vi "PicoScope6000aExampleStreamingQueue.vi"() -> ()   [LabVIEW 2010]
doc: "ps6000a Streaming example filling a single set of channel buffers at a time with LabVIEW queues."
uses:
  shared/PicoBuffers.ctl
  <vilib>/Waveform/DWDTOps.llb/DWDT Analog to Digital.vi
  PicoScope6000aLib/PicoScope6000aDigitalChannelSettings.ctl
  PicoScope6000aLib/PicoScope6000aAnalogChannelSettings.ctl
  shared/Buffer and Transfer Settings.ctl
panel:
  out "overflow":i16 format="%010b"
  in  "Channels":T1={"Channel A Settings "={"Enabled"=TRUE, "Coupling"=50, "Range"=5, "Analogue Offset"=0.0, "BandWidth"=0}, "Channel B Settings "={"Enabled"=FALSE, "Coupling"=50, "Range"=5, "Analogue Offset"=0.0, "BandWidth"=0}, "Channel C Settings "={"Enabled"=FALSE, "Coupling"=50, "Range"=5, "Analogue Offset"=0.0, "BandWidth"=0}, "Channel D Settings "={"Enabled"=FALSE, "Coupling"=50, "Range"=5, "Analogue Offset"=0.0, "BandWidth"=0}, "Channel E Settings "={"Enabled"=FALSE, "Coupling"=50, "Range"=5, "Analogue Offset"=0.0, "BandWidth"=0}, "Channel F Settings "={"Enabled"=FALSE, "Coupling"=50, "Range"=5, "Analogue Offset"=0.0, "BandWidth"=0}, "Channel G Settings "={"Enabled"=FALSE, "Coupling"=50, "Range"=5, "Analogue Offset"=0.0, "BandWidth"=0}, "Channel H Settings "={"Enabled"=FALSE, "Coupling"=50, "Range"=5, "Analogue Offset"=0.0, "BandWidth"=0}} {"Channel H Settings"."BandWidth" items=["Full"=0, "100kHz"=100000, "20kHz"=200000, "1MHz"=1000000, "20MHz"=20000000, "25MHz"=25000000, "50MHz"=50000000, "200MHz"=200000000, "250MHz"=250000000, "500MHz"=500000000]; "Channel H Settings"."Range" items=["10mV"=0, "20mV"=1, "50mV"=2, "100mV"=3, "200mV"=4, "500mV"=5, "1V"=6, "2V"=7, "5V"=8, "10V"=9, "20V"=10, "50V"=11, "100V"=12, "200V"=13, "x10_Probe_100mV"=32, "x10_Probe_200mV"=33, "x10_Probe_500mV"=34, "x10_Probe_1V"=35, "x10_Probe_2V"=36, "x10_Probe_5V"=37, "x10_Probe_10V"=38, "x10_Probe_20V"=39, "x10_Probe_50V"=40, "x10_Probe_100V"=41, "x10_Probe_200V"=42, "x10_Probe_500V"=43, "CURRENT_CLAMP_60A_2A"=10500, "CURRENT_CLAMP_60A_5A"=10501, "CURRENT_CLAMP_60A_10A"=10502, "CURRENT_CLAMP_60A_20A"=10503, "CURRENT_CLAMP_60A_50A"=10504, "CURRENT_CLAMP_60A_60A"=10505, "CURRENT_CLAMP_60A_V2_0_5A"=10600, "CURRENT_CLAMP_60A_V2_1A"=10601, "CURRENT_CLAMP_60A_V2_2A"=10602, "CURRENT_CLAMP_60A_V2_5A"=10603, "CURRENT_CLAMP_60A_V2_10A"=10604, "CURRENT_CLAMP_60A_V2_20A"=10605, "CURRENT_CLAMP_60A_V2_50A"=10606, "CURRENT_CLAMP_60A_V2_60A"=10607, "RESISTANCE_LEAD_NEG5_TO_20OHM"=7000, "RESISTANCE_LEAD_NEG50_TO_200OHM"=7001, "RESISTANCE_LEAD_NEG500_TO_2KOHM"=7002, "RESISTANCE_LEAD_NEG5K_TO_20KOHM"=7003, "RESISTANCE_LEAD_NEG50K_TO_LEAD_200KOHM"=7004, "RESISTANCE_LEAD_NEG500K_TO_LEAD_2MOHM"=7005, "RESISTANCE_LEAD_DIODE_TEST"=7006, "HT_NEG3_TO_5KV"=8950, "HT_NEG3_TO_10KV"=8951, "HT_NEG5_TO_20KV"=8952, "HT_NEG5_TO_50KV"=8953, "HT_NEG5_TO_100KV"=8954, "HT_NEG3_TO_5KV_INVERTED"=8955, "HT_NEG3_TO_10KV_INVERTED"=8956, "HT_NEG5_TO_20KV_INVERTED"=8957, "HT_NEG5_TO_50KV_INVERTED"=8958, "HT_NEG5_TO_100KV_INVERTED"=8959, "TEMPERATURE_NEG50_TO_150DEGC"=9000, "PRESSURE_SENSOR_-100k-150k_PASCALS"=9100, "PRESSURE_SENSOR_-100k_TO_400k_PASCALS"=9101, "PRESSURE_SENSOR_-200k_TO_800k_PASCALS"=9102, "PRESSURE_SENSOR_-400k_TO_1600k_PASCALS"=9103, "PRESSURE_SENSOR_-400k_TO_3400k_PASCALS"=9104, "PRESSURE_SENSOR_-150k_TO_1350k_PASCALS"=9105]; "Channel H Settings"."Coupling" items=["AC"=0, "DC 1M Ohm"=1, "DC 50 Ohm"=50]; "Channel G Settings"."BandWidth" items=["Full"=0, "100kHz"=100000, "20kHz"=200000, "1MHz"=1000000, "20MHz"=20000000, "25MHz"=25000000, "50MHz"=50000000, "200MHz"=200000000, "250MHz"=250000000, "500MHz"=500000000]; "Channel G Settings"."Range" items=["10mV"=0, "20mV"=1, "50mV"=2, "100mV"=3, "200mV"=4, "500mV"=5, "1V"=6, "2V"=7, "5V"=8, "10V"=9, "20V"=10, "50V"=11, "100V"=12, "200V"=13, "x10_Probe_100mV"=32, "x10_Probe_200mV"=33, "x10_Probe_500mV"=34, "x10_Probe_1V"=35, "x10_Probe_2V"=36, "x10_Probe_5V"=37, "x10_Probe_10V"=38, "x10_Probe_20V"=39, "x10_Probe_50V"=40, "x10_Probe_100V"=41, "x10_Probe_200V"=42, "x10_Probe_500V"=43, "CURRENT_CLAMP_60A_2A"=10500, "CURRENT_CLAMP_60A_5A"=10501, "CURRENT_CLAMP_60A_10A"=10502, "CURRENT_CLAMP_60A_20A"=10503, "CURRENT_CLAMP_60A_50A"=10504, "CURRENT_CLAMP_60A_60A"=10505, "CURRENT_CLAMP_60A_V2_0_5A"=10600, "CURRENT_CLAMP_60A_V2_1A"=10601, "CURRENT_CLAMP_60A_V2_2A"=10602, "CURRENT_CLAMP_60A_V2_5A"=10603, "CURRENT_CLAMP_60A_V2_10A"=10604, "CURRENT_CLAMP_60A_V2_20A"=10605, "CURRENT_CLAMP_60A_V2_50A"=10606, "CURRENT_CLAMP_60A_V2_60A"=10607, "RESISTANCE_LEAD_NEG5_TO_20OHM"=7000, "RESISTANCE_LEAD_NEG50_TO_200OHM"=7001, "RESISTANCE_LEAD_NEG500_TO_2KOHM"=7002, "RESISTANCE_LEAD_NEG5K_TO_20KOHM"=7003, "RESISTANCE_LEAD_NEG50K_TO_LEAD_200KOHM"=7004, "RESISTANCE_LEAD_NEG500K_TO_LEAD_2MOHM"=7005, "RESISTANCE_LEAD_DIODE_TEST"=7006, "HT_NEG3_TO_5KV"=8950, "HT_NEG3_TO_10KV"=8951, "HT_NEG5_TO_20KV"=8952, "HT_NEG5_TO_50KV"=8953, "HT_NEG5_TO_100KV"=8954, "HT_NEG3_TO_5KV_INVERTED"=8955, "HT_NEG3_TO_10KV_INVERTED"=8956, "HT_NEG5_TO_20KV_INVERTED"=8957, "HT_NEG5_TO_50KV_INVERTED"=8958, "HT_NEG5_TO_100KV_INVERTED"=8959, "TEMPERATURE_NEG50_TO_150DEGC"=9000, "PRESSURE_SENSOR_-100k-150k_PASCALS"=9100, "PRESSURE_SENSOR_-100k_TO_400k_PASCALS"=9101, "PRESSURE_SENSOR_-200k_TO_800k_PASCALS"=9102, "PRESSURE_SENSOR_-400k_TO_1600k_PASCALS"=9103, "PRESSURE_SENSOR_-400k_TO_3400k_PASCALS"=9104, "PRESSURE_SENSOR_-150k_TO_1350k_PASCALS"=9105]; "Channel G Settings"."Coupling" items=["AC"=0, "DC 1M Ohm"=1, "DC 50 Ohm"=50]; "Channel F Settings"."BandWidth" items=["Full"=0, "100kHz"=100000, "20kHz"=200000, "1MHz"=1000000, "20MHz"=20000000, "25MHz"=25000000, "50MHz"=50000000, "200MHz"=200000000, "250MHz"=250000000, "500MHz"=500000000]; "Channel F Settings"."Range" items=["10mV"=0, "20mV"=1, "50mV"=2, "100mV"=3, "200mV"=4, "500mV"=5, "1V"=6, "2V"=7, "5V"=8, "10V"=9, "20V"=10, "50V"=11, "100V"=12, "200V"=13, "x10_Probe_100mV"=32, "x10_Probe_200mV"=33, "x10_Probe_500mV"=34, "x10_Probe_1V"=35, "x10_Probe_2V"=36, "x10_Probe_5V"=37, "x10_Probe_10V"=38, "x10_Probe_20V"=39, "x10_Probe_50V"=40, "x10_Probe_100V"=41, "x10_Probe_200V"=42, "x10_Probe_500V"=43, "CURRENT_CLAMP_60A_2A"=10500, "CURRENT_CLAMP_60A_5A"=10501, "CURRENT_CLAMP_60A_10A"=10502, "CURRENT_CLAMP_60A_20A"=10503, "CURRENT_CLAMP_60A_50A"=10504, "CURRENT_CLAMP_60A_60A"=10505, "CURRENT_CLAMP_60A_V2_0_5A"=10600, "CURRENT_CLAMP_60A_V2_1A"=10601, "CURRENT_CLAMP_60A_V2_2A"=10602, "CURRENT_CLAMP_60A_V2_5A"=10603, "CURRENT_CLAMP_60A_V2_10A"=10604, "CURRENT_CLAMP_60A_V2_20A"=10605, "CURRENT_CLAMP_60A_V2_50A"=10606, "CURRENT_CLAMP_60A_V2_60A"=10607, "RESISTANCE_LEAD_NEG5_TO_20OHM"=7000, "RESISTANCE_LEAD_NEG50_TO_200OHM"=7001, "RESISTANCE_LEAD_NEG500_TO_2KOHM"=7002, "RESISTANCE_LEAD_NEG5K_TO_20KOHM"=7003, "RESISTANCE_LEAD_NEG50K_TO_LEAD_200KOHM"=7004, "RESISTANCE_LEAD_NEG500K_TO_LEAD_2MOHM"=7005, "RESISTANCE_LEAD_DIODE_TEST"=7006, "HT_NEG3_TO_5KV"=8950, "HT_NEG3_TO_10KV"=8951, "HT_NEG5_TO_20KV"=8952, "HT_NEG5_TO_50KV"=8953, "HT_NEG5_TO_100KV"=8954, "HT_NEG3_TO_5KV_INVERTED"=8955, "HT_NEG3_TO_10KV_INVERTED"=8956, "HT_NEG5_TO_20KV_INVERTED"=8957, "HT_NEG5_TO_50KV_INVERTED"=8958, "HT_NEG5_TO_100KV_INVERTED"=8959, "TEMPERATURE_NEG50_TO_150DEGC"=9000, "PRESSURE_SENSOR_-100k-150k_PASCALS"=9100, "PRESSURE_SENSOR_-100k_TO_400k_PASCALS"=9101, "PRESSURE_SENSOR_-200k_TO_800k_PASCALS"=9102, "PRESSURE_SENSOR_-400k_TO_1600k_PASCALS"=9103, "PRESSURE_SENSOR_-400k_TO_3400k_PASCALS"=9104, "PRESSURE_SENSOR_-150k_TO_1350k_PASCALS"=9105]; "Channel F Settings"."Coupling" items=["AC"=0, "DC 1M Ohm"=1, "DC 50 Ohm"=50]; "Channel E Settings"."BandWidth" items=["Full"=0, "100kHz"=100000, "20kHz"=200000, "1MHz"=1000000, "20MHz"=20000000, "25MHz"=25000000, "50MHz"=50000000, "200MHz"=200000000, "250MHz"=250000000, "500MHz"=500000000]; "Channel E Settings"."Range" items=["10mV"=0, "20mV"=1, "50mV"=2, "100mV"=3, "200mV"=4, "500mV"=5, "1V"=6, "2V"=7, "5V"=8, "10V"=9, "20V"=10, "50V"=11, "100V"=12, "200V"=13, "x10_Probe_100mV"=32, "x10_Probe_200mV"=33, "x10_Probe_500mV"=34, "x10_Probe_1V"=35, "x10_Probe_2V"=36, "x10_Probe_5V"=37, "x10_Probe_10V"=38, "x10_Probe_20V"=39, "x10_Probe_50V"=40, "x10_Probe_100V"=41, "x10_Probe_200V"=42, "x10_Probe_500V"=43, "CURRENT_CLAMP_60A_2A"=10500, "CURRENT_CLAMP_60A_5A"=10501, "CURRENT_CLAMP_60A_10A"=10502, "CURRENT_CLAMP_60A_20A"=10503, "CURRENT_CLAMP_60A_50A"=10504, "CURRENT_CLAMP_60A_60A"=10505, "CURRENT_CLAMP_60A_V2_0_5A"=10600, "CURRENT_CLAMP_60A_V2_1A"=10601, "CURRENT_CLAMP_60A_V2_2A"=10602, "CURRENT_CLAMP_60A_V2_5A"=10603, "CURRENT_CLAMP_60A_V2_10A"=10604, "CURRENT_CLAMP_60A_V2_20A"=10605, "CURRENT_CLAMP_60A_V2_50A"=10606, "CURRENT_CLAMP_60A_V2_60A"=10607, "RESISTANCE_LEAD_NEG5_TO_20OHM"=7000, "RESISTANCE_LEAD_NEG50_TO_200OHM"=7001, "RESISTANCE_LEAD_NEG500_TO_2KOHM"=7002, "RESISTANCE_LEAD_NEG5K_TO_20KOHM"=7003, "RESISTANCE_LEAD_NEG50K_TO_LEAD_200KOHM"=7004, "RESISTANCE_LEAD_NEG500K_TO_LEAD_2MOHM"=7005, "RESISTANCE_LEAD_DIODE_TEST"=7006, "HT_NEG3_TO_5KV"=8950, "HT_NEG3_TO_10KV"=8951, "HT_NEG5_TO_20KV"=8952, "HT_NEG5_TO_50KV"=8953, "HT_NEG5_TO_100KV"=8954, "HT_NEG3_TO_5KV_INVERTED"=8955, "HT_NEG3_TO_10KV_INVERTED"=8956, "HT_NEG5_TO_20KV_INVERTED"=8957, "HT_NEG5_TO_50KV_INVERTED"=8958, "HT_NEG5_TO_100KV_INVERTED"=8959, "TEMPERATURE_NEG50_TO_150DEGC"=9000, "PRESSURE_SENSOR_-100k-150k_PASCALS"=9100, "PRESSURE_SENSOR_-100k_TO_400k_PASCALS"=9101, "PRESSURE_SENSOR_-200k_TO_800k_PASCALS"=9102, "PRESSURE_SENSOR_-400k_TO_1600k_PASCALS"=9103, "PRESSURE_SENSOR_-400k_TO_3400k_PASCALS"=9104, "PRESSURE_SENSOR_-150k_TO_1350k_PASCALS"=9105]; "Channel E Settings"."Coupling" items=["AC"=0, "DC 1M Ohm"=1, "DC 50 Ohm"=50]; "Channel D Settings"."BandWidth" items=["Full"=0, "100kHz"=100000, "20kHz"=200000, "1MHz"=1000000, "20MHz"=20000000, "25MHz"=25000000, "50MHz"=50000000, "200MHz"=200000000, "250MHz"=250000000, "500MHz"=500000000]; "Channel D Settings"."Range" items=["10mV"=0, "20mV"=1, "50mV"=2, "100mV"=3, "200mV"=4, "500mV"=5, "1V"=6, "2V"=7, "5V"=8, "10V"=9, "20V"=10, "50V"=11, "100V"=12, "200V"=13, "x10_Probe_100mV"=32, "x10_Probe_200mV"=33, "x10_Probe_500mV"=34, "x10_Probe_1V"=35, "x10_Probe_2V"=36, "x10_Probe_5V"=37, "x10_Probe_10V"=38, "x10_Probe_20V"=39, "x10_Probe_50V"=40, "x10_Probe_100V"=41, "x10_Probe_200V"=42, "x10_Probe_500V"=43, "CURRENT_CLAMP_60A_2A"=10500, "CURRENT_CLAMP_60A_5A"=10501, "CURRENT_CLAMP_60A_10A"=10502, "CURRENT_CLAMP_60A_20A"=10503, "CURRENT_CLAMP_60A_50A"=10504, "CURRENT_CLAMP_60A_60A"=10505, "CURRENT_CLAMP_60A_V2_0_5A"=10600, "CURRENT_CLAMP_60A_V2_1A"=10601, "CURRENT_CLAMP_60A_V2_2A"=10602, "CURRENT_CLAMP_60A_V2_5A"=10603, "CURRENT_CLAMP_60A_V2_10A"=10604, "CURRENT_CLAMP_60A_V2_20A"=10605, "CURRENT_CLAMP_60A_V2_50A"=10606, "CURRENT_CLAMP_60A_V2_60A"=10607, "RESISTANCE_LEAD_NEG5_TO_20OHM"=7000, "RESISTANCE_LEAD_NEG50_TO_200OHM"=7001, "RESISTANCE_LEAD_NEG500_TO_2KOHM"=7002, "RESISTANCE_LEAD_NEG5K_TO_20KOHM"=7003, "RESISTANCE_LEAD_NEG50K_TO_LEAD_200KOHM"=7004, "RESISTANCE_LEAD_NEG500K_TO_LEAD_2MOHM"=7005, "RESISTANCE_LEAD_DIODE_TEST"=7006, "HT_NEG3_TO_5KV"=8950, "HT_NEG3_TO_10KV"=8951, "HT_NEG5_TO_20KV"=8952, "HT_NEG5_TO_50KV"=8953, "HT_NEG5_TO_100KV"=8954, "HT_NEG3_TO_5KV_INVERTED"=8955, "HT_NEG3_TO_10KV_INVERTED"=8956, "HT_NEG5_TO_20KV_INVERTED"=8957, "HT_NEG5_TO_50KV_INVERTED"=8958, "HT_NEG5_TO_100KV_INVERTED"=8959, "TEMPERATURE_NEG50_TO_150DEGC"=9000, "PRESSURE_SENSOR_-100k-150k_PASCALS"=9100, "PRESSURE_SENSOR_-100k_TO_400k_PASCALS"=9101, "PRESSURE_SENSOR_-200k_TO_800k_PASCALS"=9102, "PRESSURE_SENSOR_-400k_TO_1600k_PASCALS"=9103, "PRESSURE_SENSOR_-400k_TO_3400k_PASCALS"=9104, "PRESSURE_SENSOR_-150k_TO_1350k_PASCALS"=9105]; "Channel D Settings"."Coupling" items=["AC"=0, "DC 1M Ohm"=1, "DC 50 Ohm"=50]; "Channel C Settings"."BandWidth" items=["Full"=0, "100kHz"=100000, "20kHz"=200000, "1MHz"=1000000, "20MHz"=20000000, "25MHz"=25000000, "50MHz"=50000000, "200MHz"=200000000, "250MHz"=250000000, "500MHz"=500000000]; "Channel C Settings"."Range" items=["10mV"=0, "20mV"=1, "50mV"=2, "100mV"=3, "200mV"=4, "500mV"=5, "1V"=6, "2V"=7, "5V"=8, "10V"=9, "20V"=10, "50V"=11, "100V"=12, "200V"=13, "x10_Probe_100mV"=32, "x10_Probe_200mV"=33, "x10_Probe_500mV"=34, "x10_Probe_1V"=35, "x10_Probe_2V"=36, "x10_Probe_5V"=37, "x10_Probe_10V"=38, "x10_Probe_20V"=39, "x10_Probe_50V"=40, "x10_Probe_100V"=41, "x10_Probe_200V"=42, "x10_Probe_500V"=43, "CURRENT_CLAMP_60A_2A"=10500, "CURRENT_CLAMP_60A_5A"=10501, "CURRENT_CLAMP_60A_10A"=10502, "CURRENT_CLAMP_60A_20A"=10503, "CURRENT_CLAMP_60A_50A"=10504, "CURRENT_CLAMP_60A_60A"=10505, "CURRENT_CLAMP_60A_V2_0_5A"=10600, "CURRENT_CLAMP_60A_V2_1A"=10601, "CURRENT_CLAMP_60A_V2_2A"=10602, "CURRENT_CLAMP_60A_V2_5A"=10603, "CURRENT_CLAMP_60A_V2_10A"=10604, "CURRENT_CLAMP_60A_V2_20A"=10605, "CURRENT_CLAMP_60A_V2_50A"=10606, "CURRENT_CLAMP_60A_V2_60A"=10607, "RESISTANCE_LEAD_NEG5_TO_20OHM"=7000, "RESISTANCE_LEAD_NEG50_TO_200OHM"=7001, "RESISTANCE_LEAD_NEG500_TO_2KOHM"=7002, "RESISTANCE_LEAD_NEG5K_TO_20KOHM"=7003, "RESISTANCE_LEAD_NEG50K_TO_LEAD_200KOHM"=7004, "RESISTANCE_LEAD_NEG500K_TO_LEAD_2MOHM"=7005, "RESISTANCE_LEAD_DIODE_TEST"=7006, "HT_NEG3_TO_5KV"=8950, "HT_NEG3_TO_10KV"=8951, "HT_NEG5_TO_20KV"=8952, "HT_NEG5_TO_50KV"=8953, "HT_NEG5_TO_100KV"=8954, "HT_NEG3_TO_5KV_INVERTED"=8955, "HT_NEG3_TO_10KV_INVERTED"=8956, "HT_NEG5_TO_20KV_INVERTED"=8957, "HT_NEG5_TO_50KV_INVERTED"=8958, "HT_NEG5_TO_100KV_INVERTED"=8959, "TEMPERATURE_NEG50_TO_150DEGC"=9000, "PRESSURE_SENSOR_-100k-150k_PASCALS"=9100, "PRESSURE_SENSOR_-100k_TO_400k_PASCALS"=9101, "PRESSURE_SENSOR_-200k_TO_800k_PASCALS"=9102, "PRESSURE_SENSOR_-400k_TO_1600k_PASCALS"=9103, "PRESSURE_SENSOR_-400k_TO_3400k_PASCALS"=9104, "PRESSURE_SENSOR_-150k_TO_1350k_PASCALS"=9105]; "Channel C Settings"."Coupling" items=["AC"=0, "DC 1M Ohm"=1, "DC 50 Ohm"=50]; "Channel B Settings"."BandWidth" items=["Full"=0, "100kHz"=100000, "20kHz"=200000, "1MHz"=1000000, "20MHz"=20000000, "25MHz"=25000000, "50MHz"=50000000, "200MHz"=200000000, "250MHz"=250000000, "500MHz"=500000000]; "Channel B Settings"."Range" items=["10mV"=0, "20mV"=1, "50mV"=2, "100mV"=3, "200mV"=4, "500mV"=5, "1V"=6, "2V"=7, "5V"=8, "10V"=9, "20V"=10, "50V"=11, "100V"=12, "200V"=13, "x10_Probe_100mV"=32, "x10_Probe_200mV"=33, "x10_Probe_500mV"=34, "x10_Probe_1V"=35, "x10_Probe_2V"=36, "x10_Probe_5V"=37, "x10_Probe_10V"=38, "x10_Probe_20V"=39, "x10_Probe_50V"=40, "x10_Probe_100V"=41, "x10_Probe_200V"=42, "x10_Probe_500V"=43, "CURRENT_CLAMP_60A_2A"=10500, "CURRENT_CLAMP_60A_5A"=10501, "CURRENT_CLAMP_60A_10A"=10502, "CURRENT_CLAMP_60A_20A"=10503, "CURRENT_CLAMP_60A_50A"=10504, "CURRENT_CLAMP_60A_60A"=10505, "CURRENT_CLAMP_60A_V2_0_5A"=10600, "CURRENT_CLAMP_60A_V2_1A"=10601, "CURRENT_CLAMP_60A_V2_2A"=10602, "CURRENT_CLAMP_60A_V2_5A"=10603, "CURRENT_CLAMP_60A_V2_10A"=10604, "CURRENT_CLAMP_60A_V2_20A"=10605, "CURRENT_CLAMP_60A_V2_50A"=10606, "CURRENT_CLAMP_60A_V2_60A"=10607, "RESISTANCE_LEAD_NEG5_TO_20OHM"=7000, "RESISTANCE_LEAD_NEG50_TO_200OHM"=7001, "RESISTANCE_LEAD_NEG500_TO_2KOHM"=7002, "RESISTANCE_LEAD_NEG5K_TO_20KOHM"=7003, "RESISTANCE_LEAD_NEG50K_TO_LEAD_200KOHM"=7004, "RESISTANCE_LEAD_NEG500K_TO_LEAD_2MOHM"=7005, "RESISTANCE_LEAD_DIODE_TEST"=7006, "HT_NEG3_TO_5KV"=8950, "HT_NEG3_TO_10KV"=8951, "HT_NEG5_TO_20KV"=8952, "HT_NEG5_TO_50KV"=8953, "HT_NEG5_TO_100KV"=8954, "HT_NEG3_TO_5KV_INVERTED"=8955, "HT_NEG3_TO_10KV_INVERTED"=8956, "HT_NEG5_TO_20KV_INVERTED"=8957, "HT_NEG5_TO_50KV_INVERTED"=8958, "HT_NEG5_TO_100KV_INVERTED"=8959, "TEMPERATURE_NEG50_TO_150DEGC"=9000, "PRESSURE_SENSOR_-100k-150k_PASCALS"=9100, "PRESSURE_SENSOR_-100k_TO_400k_PASCALS"=9101, "PRESSURE_SENSOR_-200k_TO_800k_PASCALS"=9102, "PRESSURE_SENSOR_-400k_TO_1600k_PASCALS"=9103, "PRESSURE_SENSOR_-400k_TO_3400k_PASCALS"=9104, "PRESSURE_SENSOR_-150k_TO_1350k_PASCALS"=9105]; "Channel B Settings"."Coupling" items=["AC"=0, "DC 1M Ohm"=1, "DC 50 Ohm"=50]; "Channel A Settings"."Range" items=["10mV"=0, "20mV"=1, "50mV"=2, "100mV"=3, "200mV"=4, "500mV"=5, "1V"=6, "2V"=7, "5V"=8, "10V"=9, "20V"=10, "50V"=11, "100V"=12, "200V"=13, "x10_Probe_100mV"=32, "x10_Probe_200mV"=33, "x10_Probe_500mV"=34, "x10_Probe_1V"=35, "x10_Probe_2V"=36, "x10_Probe_5V"=37, "x10_Probe_10V"=38, "x10_Probe_20V"=39, "x10_Probe_50V"=40, "x10_Probe_100V"=41, "x10_Probe_200V"=42, "x10_Probe_500V"=43, "CURRENT_CLAMP_60A_2A"=10500, "CURRENT_CLAMP_60A_5A"=10501, "CURRENT_CLAMP_60A_10A"=10502, "CURRENT_CLAMP_60A_20A"=10503, "CURRENT_CLAMP_60A_50A"=10504, "CURRENT_CLAMP_60A_60A"=10505, "CURRENT_CLAMP_60A_V2_0_5A"=10600, "CURRENT_CLAMP_60A_V2_1A"=10601, "CURRENT_CLAMP_60A_V2_2A"=10602, "CURRENT_CLAMP_60A_V2_5A"=10603, "CURRENT_CLAMP_60A_V2_10A"=10604, "CURRENT_CLAMP_60A_V2_20A"=10605, "CURRENT_CLAMP_60A_V2_50A"=10606, "CURRENT_CLAMP_60A_V2_60A"=10607, "RESISTANCE_LEAD_NEG5_TO_20OHM"=7000, "RESISTANCE_LEAD_NEG50_TO_200OHM"=7001, "RESISTANCE_LEAD_NEG500_TO_2KOHM"=7002, "RESISTANCE_LEAD_NEG5K_TO_20KOHM"=7003, "RESISTANCE_LEAD_NEG50K_TO_LEAD_200KOHM"=7004, "RESISTANCE_LEAD_NEG500K_TO_LEAD_2MOHM"=7005, "RESISTANCE_LEAD_DIODE_TEST"=7006, "HT_NEG3_TO_5KV"=8950, "HT_NEG3_TO_10KV"=8951, "HT_NEG5_TO_20KV"=8952, "HT_NEG5_TO_50KV"=8953, "HT_NEG5_TO_100KV"=8954, "HT_NEG3_TO_5KV_INVERTED"=8955, "HT_NEG3_TO_10KV_INVERTED"=8956, "HT_NEG5_TO_20KV_INVERTED"=8957, "HT_NEG5_TO_50KV_INVERTED"=8958, "HT_NEG5_TO_100KV_INVERTED"=8959, "TEMPERATURE_NEG50_TO_150DEGC"=9000, "PRESSURE_SENSOR_-100k-150k_PASCALS"=9100, "PRESSURE_SENSOR_-100k_TO_400k_PASCALS"=9101, "PRESSURE_SENSOR_-200k_TO_800k_PASCALS"=9102, "PRESSURE_SENSOR_-400k_TO_1600k_PASCALS"=9103, "PRESSURE_SENSOR_-400k_TO_3400k_PASCALS"=9104, "PRESSURE_SENSOR_-150k_TO_1350k_PASCALS"=9105]; "Channel A Settings"."BandWidth" items=["Full"=0, "100kHz"=100000, "20kHz"=200000, "1MHz"=1000000, "20MHz"=20000000, "25MHz"=25000000, "50MHz"=50000000, "200MHz"=200000000, "250MHz"=250000000, "500MHz"=500000000]; "Channel A Settings"."Coupling" items=["AC"=0, "DC 1M Ohm"=1, "DC 50 Ohm"=50]}
  out "Triggered":bool
  out "triggerAt":u64
  in  "Poll Delay %":dbl=1.0 format="%#_13g"
  in  "Poll Holdoff %":dbl=33.0 format="%#_13g"
  out "Port 0":digitalwaveform(graph)={"t0"=timestamp(0 s since 1904-01-01), "dt"=1.004800013071339e-06, "Y"={"transitions"=[], "data"=[]}}
  out "Analog Channels":cluster{i32, dbl, "Data":dbl[]}[](graph)
  in  "Write to TDMS file":bool
  out "Queue depth":i32(graph)
  out "queue depth":i32
  in  "Data file":path=path "PicoScope6000aExampleStreaming Data"
  out "Max ADC value":i16
  out "DownSample Interval (sec)":dbl=1.0000000130088963e-06 format="%#.5p"
  out "Chunk time":u32
  out "Elapsed time":dbl
  in  "Auto Stop":bool
  in  "Apply Settings":bool
  in  "Digital Channels":T2={"Port 0 Settings "={"Enabled"=FALSE, "Hysteresis"=3, "Threshold Level (Volts)"=[1.0, 1.0, 1.0, 1.0, 1.0, 1.0, 1.0, 1.0]}, "Port 1 Settings"={"Enabled"=FALSE, "Hysteresis"=3, "Threshold Level (Volts)"=[1.0, 1.0, 1.0, 1.0, 1.0, 1.0, 1.0, 1.0]}} {"Port 1 Settings"."Threshold Level (Volts)" format="%#_4p"; "Port 1 Settings"."Hysteresis" items=["PICO_VERY_HIGH_400MV", "PICO_HIGH_200MV", "PICO_NORMAL_100MV", "PICO_LOW_50MV"]; "Port 0 Settings"."Threshold Level (Volts)" format="%#_4p"; "Port 0 Settings"."Hysteresis" items=["PICO_VERY_HIGH_400MV", "PICO_HIGH_200MV", "PICO_NORMAL_100MV", "PICO_LOW_50MV"]}
  in  "No of Buffers":i32=2 min=2
  in  "Streaming Acquisition Settings":T3={"preTriggerSamples"=0, "postTriggerSamples"=1000000, "Requested sampleInterval"=100.0, "sampleIntervalTimeUnits"=2} {"sampleIntervalTimeUnits" items=["femtoseconds", "picoseconds", "nanoseconds", "microseconds", "millseconds", "seconds"]; "postTriggerSamples" format="%_6p"; "preTriggerSamples" format="%_6p"}
  in  "Buffer and Transfer Settings":T4={"startIndex"=0, "Samples"=1000000, "Down Sample Ratio"=1, "Down-Sample Mode"=2147483648} {"Down-Sample Mode" items=["RAW none"=2147483648, "None"=0, "Aggregate"=1, "Decimate"=2, "Average"=4]; "Down Sample Ratio" step=1; "Samples" format="%_6p"}
  in  "Trigger Settings":T5={"Trigger Enabled"=FALSE, "Trigger Threshold (Volts)"=0.0, "Trigger Direction"=2, "Trigger Delay (samples)"=0, "Auto Trigger Time (us)"=100000, "Trigger Source"=0} {"Trigger Source" items=["Channel A"=0, "Channel B"=1, "Channel C"=2, "Channel D"=3, "Channel E"=4, "Channel F"=5, "Channel G"=6, "Channel H"=7, "Port 0"=128, "Port 1"=129, "Trigger AUX"=1001]; "Trigger Direction" items=["Rising"=2, "Falling"=3]; "Trigger Threshold (Volts)" format="%#_6p"}
  in  "stop":bool
  out "Device Info":T6
  out "Pico 6000a Units":string
  in  "Resolution":u32(ring) items=["8-bit"=0, "12-bit"=1, "14-bit"=2, "15-bit"=3, "16-bit"=4, "10-bit"=10]
  in  "Serial Number":string
  in  "Use Serial Number":bool
  in  "error in (no error)":errorcluster
  # "LSB ChA"
  # "D8-D15"
  # "DO-D7"
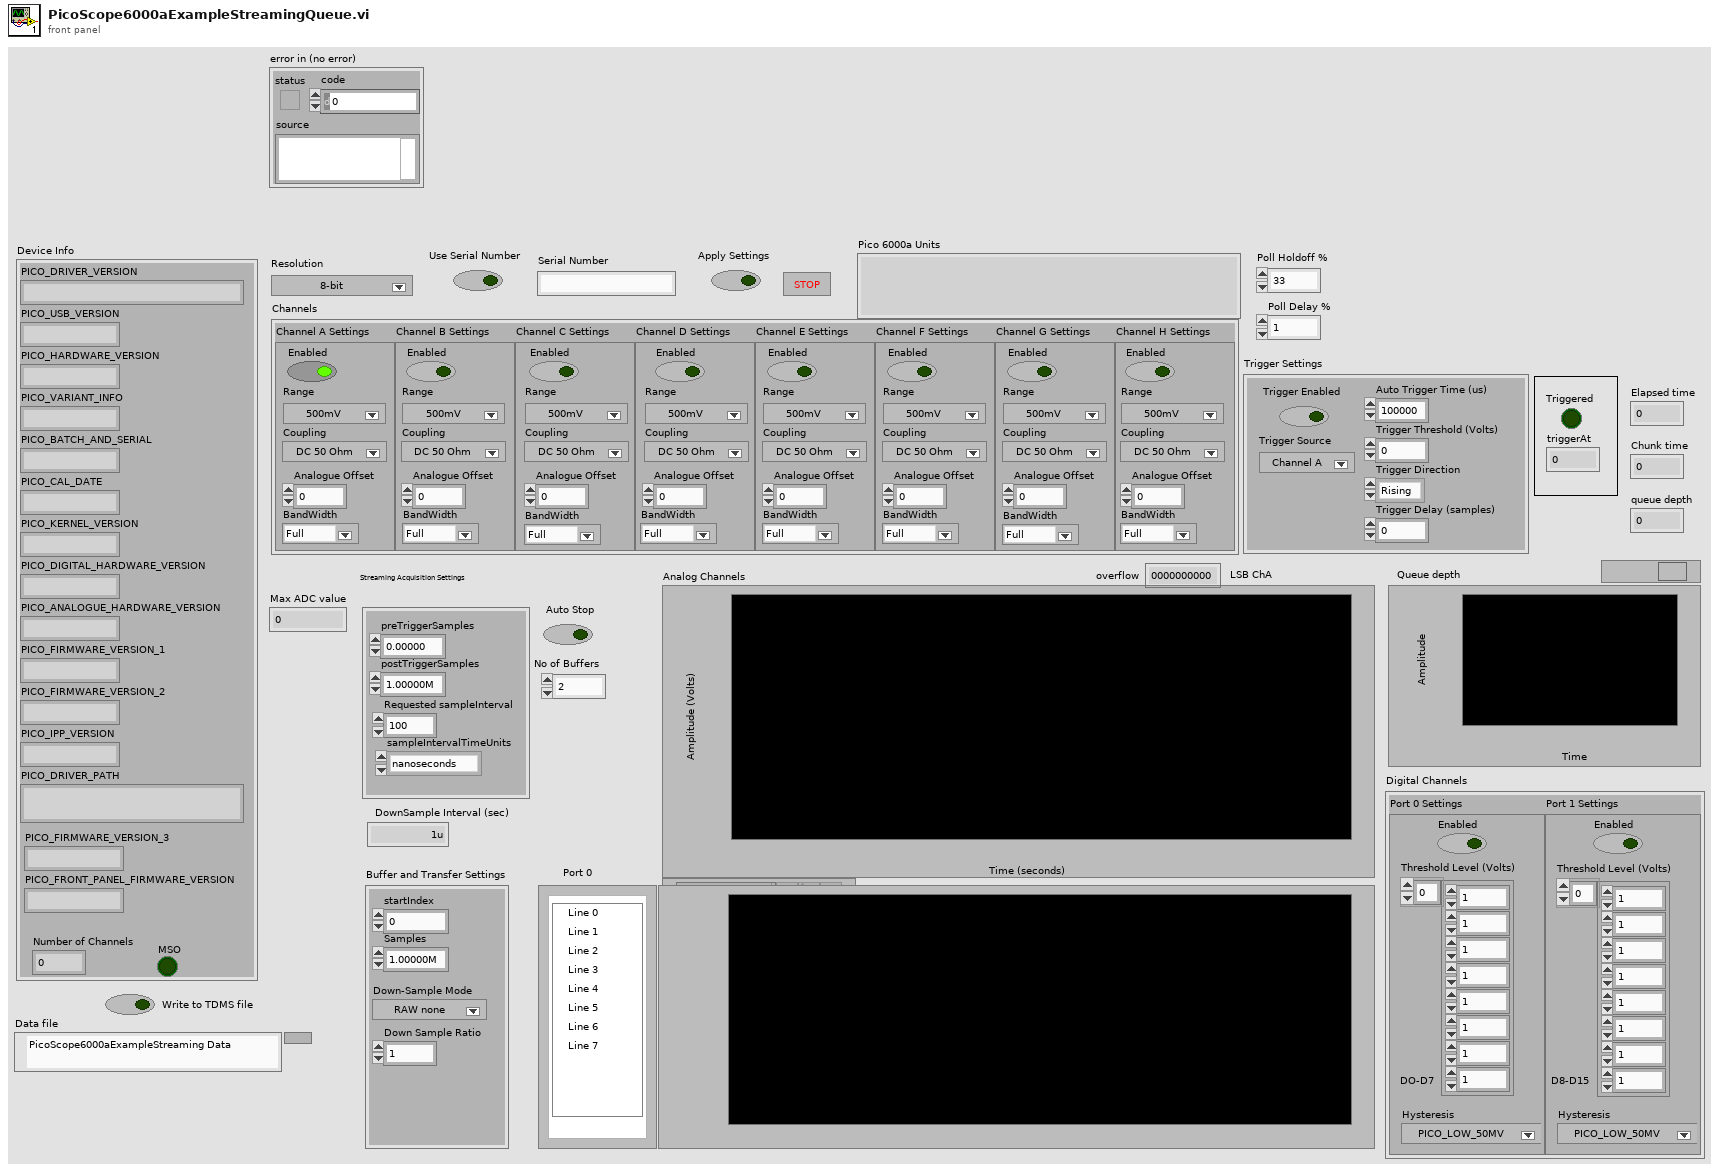
[diagram p1: front panel]
types:
  T1 = typedef "PicoScope6000aAnalogChannelSettings.ctl" = cluster{"Channel A Settings ":cluster{"Enabled":bool, "Coupling":i16, "Range":u32, "Analogue Offset":dbl, "BandWidth":u32}, "Channel B Settings ":cluster{"Enabled":bool, "Coupling":i16, "Range":u32, "Analogue Offset":dbl, "BandWidth":u32}, "Channel C Settings ":cluster{"Enabled":bool, "Coupling":i16, "Range":u32, "Analogue Offset":dbl, "BandWidth":u32}, "Channel D Settings ":cluster{"Enabled":bool, "Coupling":i16, "Range":u32, "Analogue Offset":dbl, "BandWidth":u32}, "Channel E Settings ":cluster{"Enabled":bool, "Coupling":i16, "Range":u32, "Analogue Offset":dbl, "BandWidth":u32}, "Channel F Settings ":cluster{"Enabled":bool, "Coupling":i16, "Range":u32, "Analogue Offset":dbl, "BandWidth":u32}, "Channel G Settings ":cluster{"Enabled":bool, "Coupling":i16, "Range":u32, "Analogue Offset":dbl, "BandWidth":u32}, "Channel H Settings ":cluster{"Enabled":bool, "Coupling":i16, "Range":u32, "Analogue Offset":dbl, "BandWidth":u32}}
  T2 = typedef "PicoScope6000aDigitalChannelSettings.ctl" = cluster{"Port 0 Settings ":cluster{"Enabled":bool, "Hysteresis":u32, "Threshold Level (Volts)":dbl[]}, "Port 1 Settings":cluster{"Enabled":bool, "Hysteresis":u32, "Threshold Level (Volts)":dbl[]}}
  T3 = cluster{"preTriggerSamples":u64, "postTriggerSamples":u64, "Requested sampleInterval":dbl, "sampleIntervalTimeUnits":u32}
  T4 = typedef "Buffer and Transfer Settings.ctl" = cluster{"startIndex":u64, "Samples":u64, "Down Sample Ratio":u64, "Down-Sample Mode":u32}
  T5 = cluster{"Trigger Enabled":bool, "Trigger Threshold (Volts)":dbl, "Trigger Direction":u16, "Trigger Delay (samples)":u64, "Auto Trigger Time (us)":u32, "Trigger Source":u32}
  T6 = cluster{"PICO_DRIVER_VERSION":string, "PICO_USB_VERSION":string, "PICO_HARDWARE_VERSION":string, "PICO_VARIANT_INFO":string, "PICO_BATCH_AND_SERIAL":string, "PICO_CAL_DATE":string, "PICO_KERNEL_VERSION":string, "PICO_DIGITAL_HARDWARE_VERSION":string, "PICO_ANALOGUE_HARDWARE_VERSION":string, "PICO_FIRMWARE_VERSION_1":string, "PICO_FIRMWARE_VERSION_2":string, "PICO_IPP_VERSION":string, "PICO_DRIVER_PATH":string, "PICO_FIRMWARE_VERSION_3":string, "PICO_FRONT_PANEL_FIRMWARE_VERSION":string, "Number of Channels":i16, "MSO":bool}
  T7 = typedef "PicoBuffers.ctl" = cluster{"Max Buffer Pointers":u64[][][], "Min Buffer Pointers":u64[][][], "StreamingDataInfo":cluster{"Channel":u32, "Down-Sample Mode":u32, "PICO_DATA_TYPE":enum32{"PICO_INT8_T", "PICO_INT16_T", "PICO_INT32_T", "PICO_UINT32_T", "PICO_INT64_T", ""}, "Samples":i32, "bufferIndex":u64, "startIndex":i32, "overflow":i16}[][]}
  T8 = enum16{"open", "open or create", "create or replace", "create", "open (read-only)"}
  T9 = cluster{"sampleInterval":dbl, "sampleIntervalTimeUnits":u32}
  T10 = cluster{"triggerAt":u64, "triggered":bool, "autoStop":bool}
  T11 = cluster{"Channel A Buffer":i16[], "Channel B Buffer":i16[], "Channel C Buffer":i16[], "Channel D Buffer":i16[], "Channel E Buffer":i16[], "Channel F Buffer":i16[], "Channel G Buffer":i16[], "Channel H Buffer":i16[], "Port 0 Buffer":i16[], "Port 1 Buffer":i16[]}
  T12 = cluster{"Channel":u32, "Down-Sample Mode":u32, "PICO_DATA_TYPE":enum32{"PICO_INT8_T", "PICO_INT16_T", "PICO_INT32_T", "PICO_UINT32_T", "PICO_INT64_T", ""}, "Samples":i32, "bufferIndex":u64, "startIndex":i32, "overflow":i16}[][]
  T13 = cluster{"Channel":u32, "Down-Sample Mode":u32, "PICO_DATA_TYPE":enum32{"PICO_INT8_T", "PICO_INT16_T", "PICO_INT32_T", "PICO_UINT32_T", "PICO_INT64_T", ""}, "Samples":i32, "bufferIndex":u64, "startIndex":i32, "overflow":i16}[]
  T14 = cluster{"Channel":u32, "Down-Sample Mode":u32, "PICO_DATA_TYPE":enum32{"PICO_INT8_T", "PICO_INT16_T", "PICO_INT32_T", "PICO_UINT32_T", "PICO_INT64_T", ""}, "Samples":i32, "bufferIndex":u64, "startIndex":i32, "overflow":i16}
  T15 = cluster{i32, "DownSample Interval (sec)":dbl, "Data":dbl[]}
  T16 = cluster{i32, "DownSample Interval (sec)":dbl, "Data":dbl[]}[]
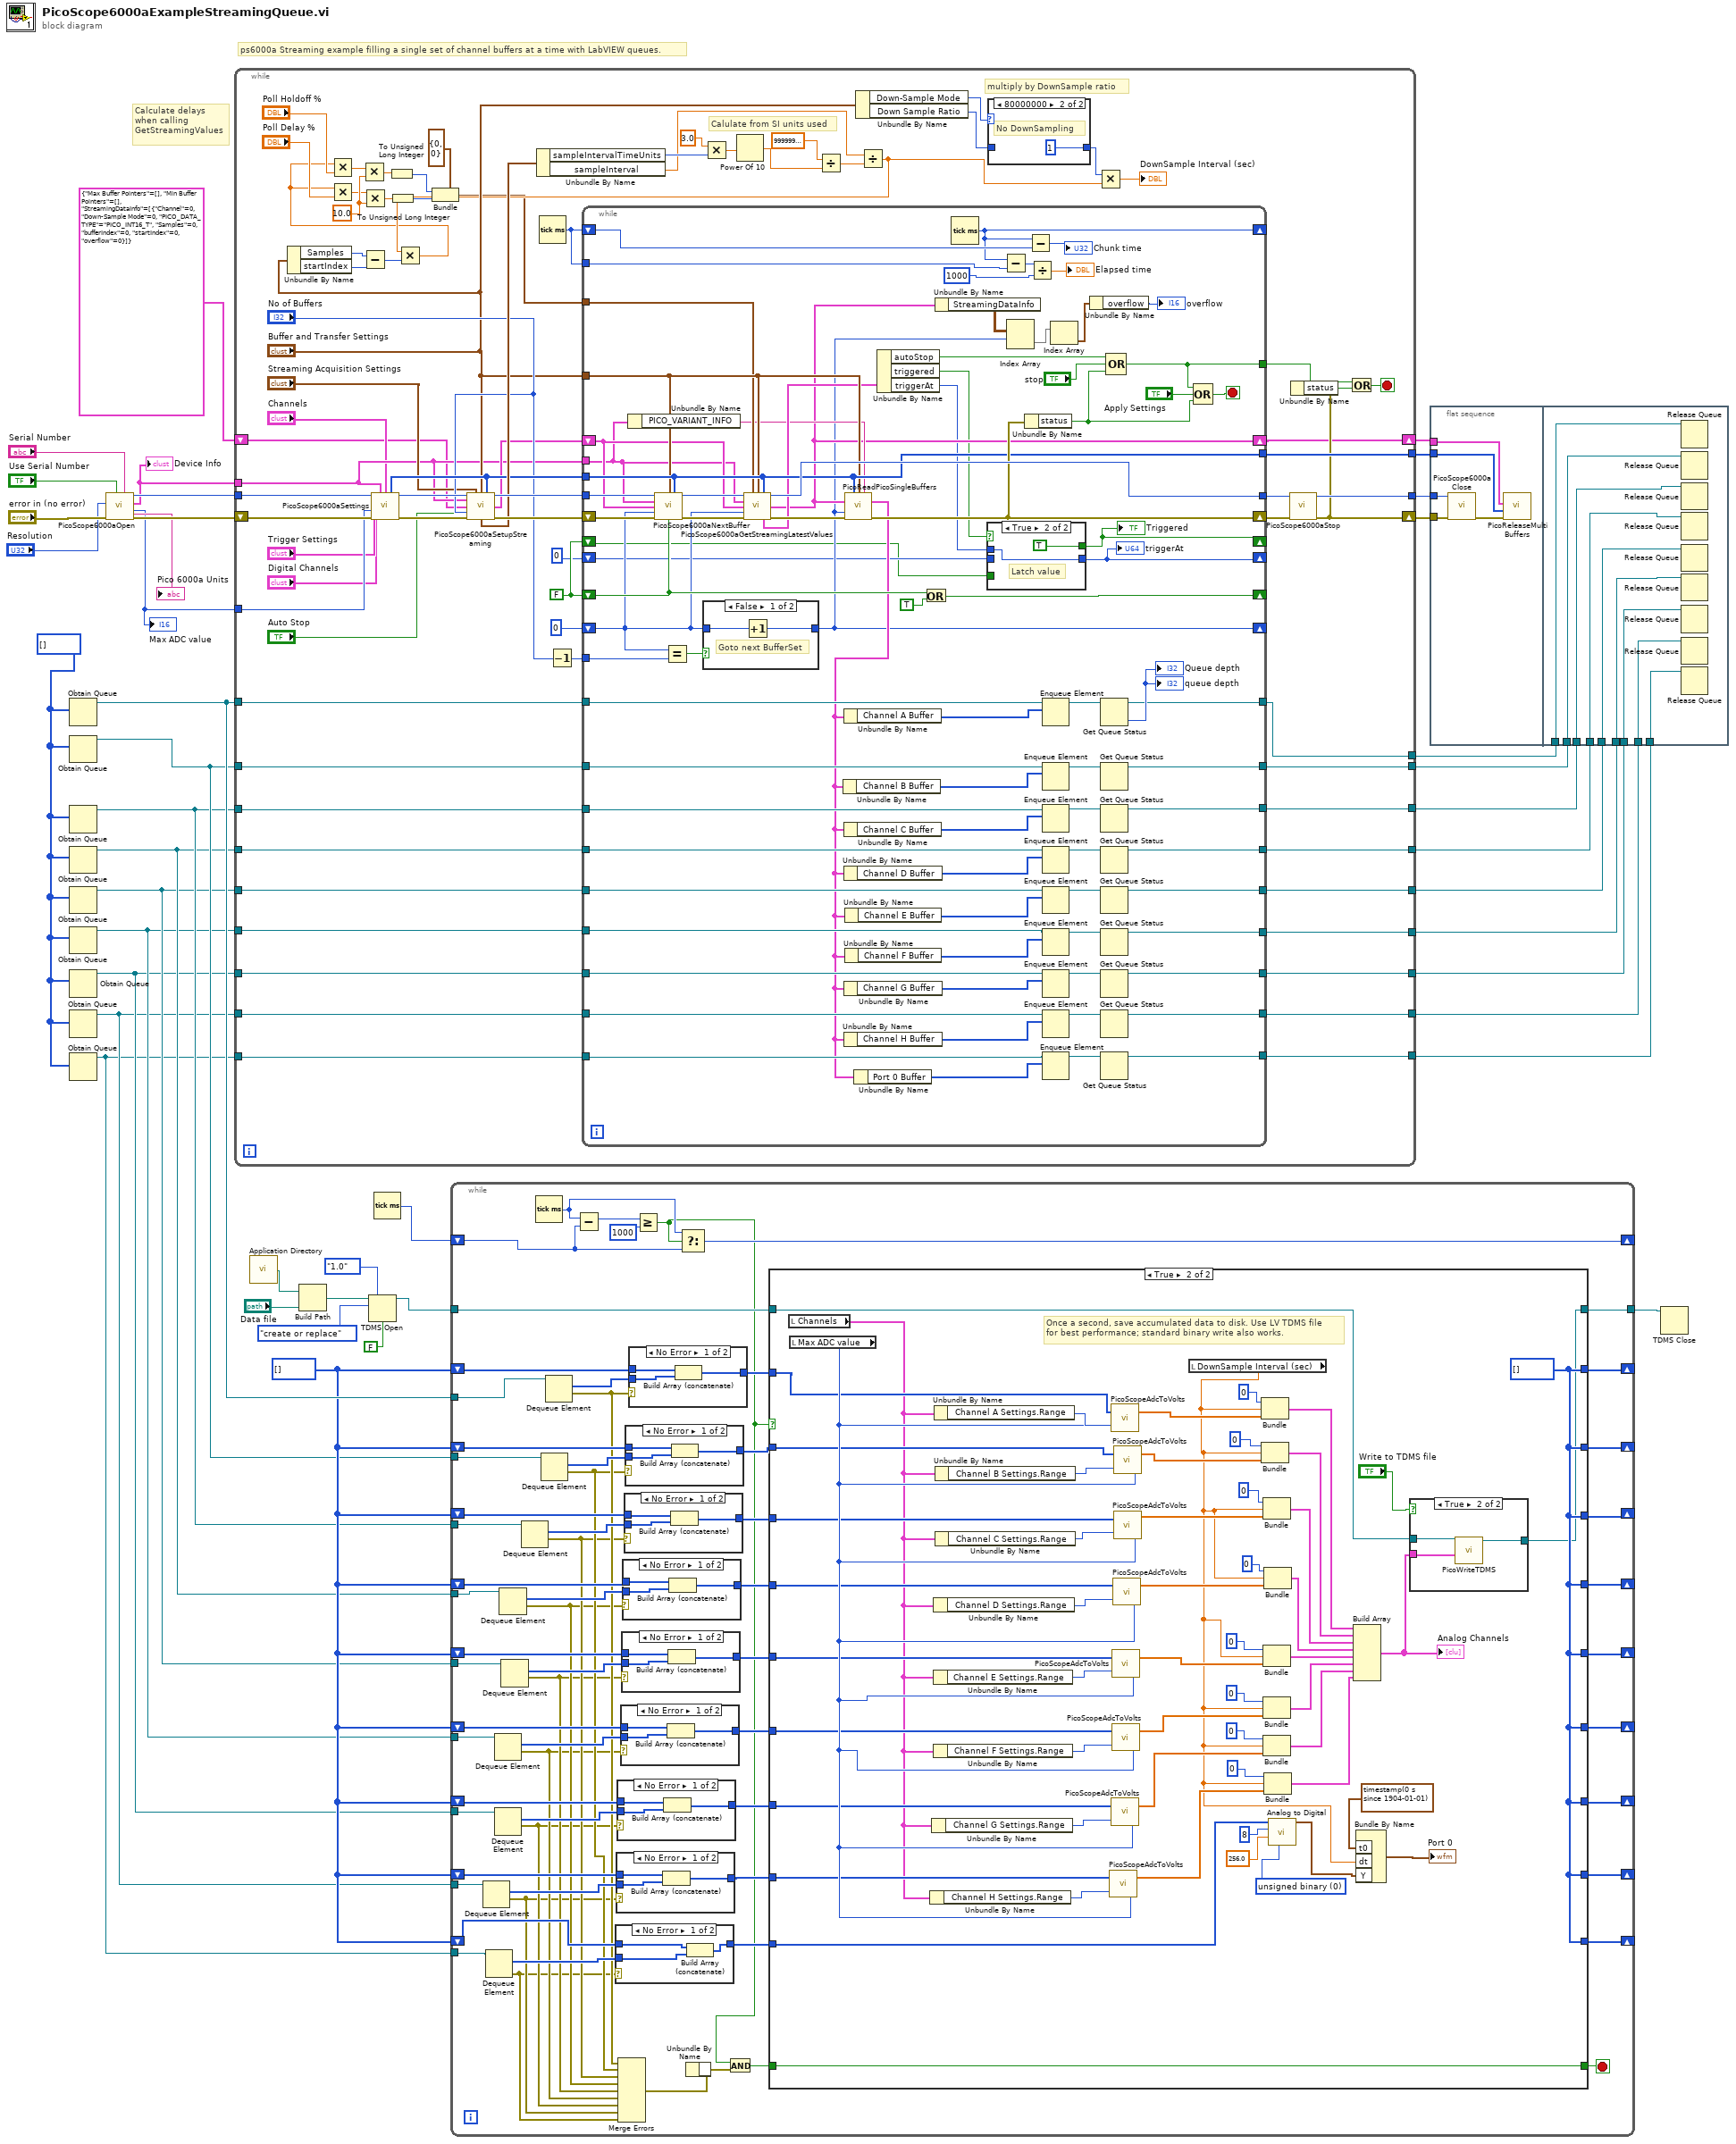
[diagram p0: block diagram]
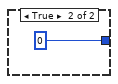
[diagram p14: hidden frame]
diagram:
  w17 = i16[] [] ("History Data")
  w18 = i16[] [] ("History Data")
  # "Calculate delays\nwhen calling\nGetStreamingValues"
  # "ps6000a Streaming example filling a single set of channel buffers at a time with LabVIEW queues."
  n1 = Obtain Queue(element data type=w17) -> (queue out=w20:refnum<queue>)  [unwired: 4 in, 2 out]
  n2 = Obtain Queue(element data type=w17) -> (queue out=w16:refnum<queue>)  [unwired: 4 in, 2 out]
  n3 = Obtain Queue(element data type=w17) -> (queue out=w15:refnum<queue>)  [unwired: 4 in, 2 out]
  n4 = Obtain Queue(element data type=w17) -> (queue out=w14:refnum<queue>)  [unwired: 4 in, 2 out]
  n5 = Obtain Queue(element data type=w17) -> (queue out=w13:refnum<queue>)  [unwired: 4 in, 2 out]
  n6 = Obtain Queue(element data type=w17) -> (queue out=w12:refnum<queue>)  [unwired: 4 in, 2 out]
  n7 = Obtain Queue(element data type=w17) -> (queue out=w11:refnum<queue>)  [unwired: 4 in, 2 out]
  n8 = Obtain Queue(element data type=w17) -> (queue out=w10:refnum<queue>)  [unwired: 4 in, 2 out]
  n9 = Obtain Queue(element data type=w17) -> (queue out=w9:refnum<queue>)  [unwired: 4 in, 2 out]
  n10 = call "PicoScope6000aOpen.vi"("Serial Number"="Serial Number", "Use Serial Number"="Use Serial Number", "error in (no error)"="error in (no error)", "Resolution"="Resolution") -> ("error out"=w39:errorcluster, "Max ADC value"=w26:i16, "Device Info"=w36:T6, "handle out"=w40:i16, "Pico 6000a Units"=→"Pico 6000a Units":string)  [unwired: 2 in, 1 out]
  "Device Info" <- w36
  "Max ADC value" <- w26
  n11 = while {
    tunnel: w40 -> [w121]
    tunnel: [w92] -> w23
    tunnel: w36 -> [w50]
    tunnel: w26 -> [w119]
    tunnel: [w104] -> w25
    shift-right: [w91] -> w24
    shift-left: w39 -> [w120]
    tunnel: w20 -> [w86]
    tunnel: w16 -> [w85]
    tunnel: [w84] -> w22
    tunnel: [w83] -> w21
    tunnel: w15 -> [w82]
    tunnel: w14 -> [w81]
    tunnel: w13 -> [w80]
    tunnel: w12 -> [w79]
    tunnel: w11 -> [w78]
    tunnel: w10 -> [w77]
    tunnel: w9 -> [w76]
    tunnel: [w75] -> w8
    tunnel: [w74] -> w7
    tunnel: [w73] -> w6
    tunnel: [w72] -> w5
    tunnel: [w71] -> w4
    tunnel: [w70] -> w3
    tunnel: [w69] -> w2
    shift-right: [w46] -> w1
    shift-left: T7 {"Max Buffer Pointers"=[], "Min Buffer Pointers"=[], "StreamingDataInfo"=[[{"Channel"=0, "Down-Sample Mode"=0, "PICO_DATA_TYPE"=enum."PICO_INT16_T", "Samples"=0, "bufferIndex"=0, "startIndex"=0, "overflow"=0}]]} ("Data Pointers") -> [w47]
    stop <- w99 stop-if-true
    w60 = 10.0 ("y")
    w45 = FALSE ("SetDataBuffer0")
    # "Calulate from SI units used"
    # "multiply by DownSample ratio"
    n12 = Unbundle By Name("Buffer and Transfer Settings") -> ("Samples"=w52:u64, "startIndex"=w53:u64)
    n13 = Subtract(x=w52, y=w53) -> (x-y=w51:u64)
    n14 = call "PicoScope6000aSettings.vi"("handle in"=w121, "Device Info"=w50, "Channels"="Channels", "Max ADC value"=w119, "error in (no error)"=w120, "Trigger Settings"="Trigger Settings", "Digital Channels"="Digital Channels") -> ("Enabled array"=w102:i16[], "handle out"=w115:i16, "error out"=w116:errorcluster)  [unwired: 6 in]
    n15 = call "PicoScope6000aSetupStreaming.vi"("handle in"=w115, "Streaming Acquisition Settings"="Streaming Acquisition Settings", "Buffer and Transfer Settings"="Buffer and Transfer Settings", "enabled array"=w102, "Device Info"=w50, "Data Pointers In"=w47, "Number of Buffers"="No of Buffers", "error in (no error)"=w116, "Auto Stop"="Auto Stop") -> ("handle out"=w108:i16, "Data Pointers"=w97:T7, "Actual sampleInterval"=w106:T9, "error out"=w107:errorcluster)  [unwired: 3 in]
    n16 = Unbundle By Name(w106) -> ("sampleIntervalTimeUnits"=w111:u32, "sampleInterval"=w105:dbl)
    n17 = Tick Count (ms)() -> (millisecond timer value=w49:u32)
    n18 = Decrement(x="No of Buffers") -> (x-1=w87:i32)
    n19 = Multiply(x=3.0, y=w111) -> (x*y=w112:dbl)
    n20 = Power Of 10(x=w112) -> (10^x=w110:dbl)
    n21 = Divide(x=sgl 1000000000000000.0 ("y"), y=w110) -> (x/y=w109:dbl)
    n22 = Unbundle By Name("Buffer and Transfer Settings") -> ("Down-Sample Mode"=w93:u32, "Down Sample Ratio"=w94:u64)
    n23 = Divide(x=w105, y=w109) -> (x/y=w66:dbl)
    n24 = Multiply(x=w66, y=w51) -> (x*y=w54:dbl)
    n25 = Multiply(x=w54, y="Poll Holdoff %") -> (x*y=w58:dbl)
    n26 = Multiply(x=w54, y="Poll Delay %") -> (x*y=w59:dbl)
    n27 = Multiply(x=w58, y=w60) -> (x*y=w63:dbl)
    n28 = Multiply(x=w59, y=w60) -> (x*y=w64:dbl)
    n29 = To Unsigned Long Integer(number=w63) -> (unsigned 32bit integer=w61:u32)
    n30 = To Unsigned Long Integer(number=w64) -> (unsigned 32bit integer=w62:u32)
    n31 = Bundle(cluster=cluster{u32, u32} {0, 0}, w61, w62) -> (w65:cluster{u32, u32})
    n32 = while {
      tunnel: "Buffer and Transfer Settings" -> [w189]
      tunnel: w108 -> [w196]
      tunnel: w102 -> [w190]
      tunnel: [w192] -> w89
      shift-right: [w191] -> w90
      shift-left: w107 -> [w197]
      shift-right: [w203] -> _
      shift-left: w45 -> [w188]
      tunnel: [w190] -> w104
      tunnel: [w199] -> w100
      tunnel: w50 -> [w136]
      tunnel: w65 -> [w138]
      shift-right: [w132] -> _
      shift-left: 0 ("No of Buffers") -> [w185]
      shift-right: [w134] -> w46
      shift-left: w97 -> [w187]
      tunnel: w87 -> [w183]
      shift-right: [w177] -> _
      shift-left: w49 -> [w178]
      tunnel: w86 -> [w173]
      tunnel: w85 -> [w172]
      tunnel: [w171] -> w84
      tunnel: [w170] -> w83
      tunnel: w82 -> [w163]
      tunnel: w81 -> [w162]
      tunnel: w80 -> [w161]
      tunnel: w79 -> [w159]
      tunnel: w78 -> [w158]
      tunnel: w77 -> [w157]
      tunnel: w76 -> [w156]
      tunnel: [w155] -> w75
      tunnel: [w154] -> w74
      tunnel: [w153] -> w73
      tunnel: [w152] -> w72
      tunnel: [w151] -> w71
      tunnel: [w150] -> w70
      tunnel: [w149] -> w69
      tunnel: w49 -> [w135]
      shift-right: [w130] -> _
      shift-left: w45 -> [w126]
      shift-right: [w125] -> _
      shift-left: u64 0 ("triggerAt") -> [w129]
      stop <- w202 stop-if-true
      n33 = Unbundle By Name(w136) -> ("PICO_VARIANT_INFO"=w137:string)
      n34 = call "PicoScope6000aNextBuffer.vi"("handle in"=w196, "Buffer and Transfer Settings"=w189, "enabled array"=w190, "Device Info"=w136, "Data Pointers In"=w187, "Buffer Number"=w185, "error in (no error)"=w197, "LoopFlag"=w188) -> ("handle out"=w193:i16, "error out"=w195:errorcluster)  [unwired: 6 in]
      n35 = Equal?(x=w185, y=w183) -> (x = y?=w186:bool)
      n36 = case shown="False" w186 {
        tunnel: w185 -> [w210 _]
        tunnel: [w209 0] -> w132
        frame False {
          # "Goto next BufferSet"
          n37 = Increment(x=w210) -> (x+1=w209:i32)
        }
        frame True {
        }
      }
      n38 = call "PicoScope6000aGetStreamingLatestValues.vi"("handle in"=w193, "Polling Delays ms"=w138, "Buffer and Transfer Settings"=w189, "enabled array"=w190, "Device Info"=w136, "Data Pointers In"=w187, "Buffer number"=w185, "error in (no error)"=w195) -> ("handle out"=w192:i16, "Data Pointers Out"=w134:T7, "tPicoStreamingDataTriggerInfo"=w184:T10, "error out"=w194:errorcluster)  [unwired: 4 in]
      n39 = call "PicoReadPicoSingleBuffers.vi"("enabled array"=w190, "Buffer and Transfer Settings"=w189, "Variant"=w137, "Data Pointers"=w134, "Buffer Number"=w132, "error in (no error)"=w194) -> ("MaxBuffers (Max or non-aggregated)"=w140:T11, "error out"=w191:errorcluster)  [unwired: 7 in, 1 out]
      n40 = Unbundle By Name(w140) -> ("Channel B Buffer"=w148:i16[])
      n41 = Unbundle By Name(w140) -> ("Channel A Buffer"=w139:i16[])
      n42 = Unbundle By Name(w140) -> ("Channel C Buffer"=w147:i16[])
      n43 = Unbundle By Name(w140) -> ("Channel D Buffer"=w146:i16[])
      n44 = Unbundle By Name(w140) -> ("Channel G Buffer"=w143:i16[])
      n45 = Unbundle By Name(w140) -> ("Channel H Buffer"=w142:i16[])
      n46 = Unbundle By Name(w140) -> ("Channel E Buffer"=w145:i16[])
      n47 = Unbundle By Name(w140) -> ("Channel F Buffer"=w144:i16[])
      n48 = Unbundle By Name(w140) -> ("Port 0 Buffer"=w141:i16[])
      n49 = Unbundle By Name(w184) -> ("autoStop"=w131:bool, "triggered"=w127:bool, "triggerAt"=w128:u64)
      n50 = Or(x=w188, y=TRUE) -> (x .or. y?=w203:bool)
      n51 = Unbundle By Name(w134) -> ("StreamingDataInfo"=w133:T12)
      n52 = Tick Count (ms)() -> (millisecond timer value=w177:u32)
      n53 = case shown="True" w127 {
        tunnel: [w206 TRUE] -> w130
        tunnel: [w205 w207] -> w125
        tunnel: w129 -> [w205 _]
        tunnel: w128 -> [_ w207]
        tunnel: w126 -> [w206 _]
        frame False {
        }
        frame True {
          # "Latch value"
        }
      }
      "Triggered" <- w130
      "triggerAt" <- w125
      n54 = Subtract(x=w177, y=w135) -> (x-y=w180:u32)
      n55 = Index Array(array=w133, index (row)=w132) -> (element=w124:T13)  [unwired: 1 in]
      n56 = Unbundle By Name(w191) -> ("status"=w198:bool)
      n57 = Subtract(x=w177, y=w178) -> (x-y=→"Chunk time":u32)
      n58 = Divide(x=w180, y=u32 1000) -> (x/y=→"Elapsed time":dbl)
      n59 = Enqueue Element(queue=w173, element=w139) -> (queue out=w175:refnum<queue>)  [unwired: 2 in, 2 out]
      n60 = Enqueue Element(queue=w172, element=w148) -> (queue out=w174:refnum<queue>)  [unwired: 2 in, 2 out]
      n61 = Enqueue Element(queue=w163, element=w147) -> (queue out=w169:refnum<queue>)  [unwired: 2 in, 2 out]
      n62 = Enqueue Element(queue=w162, element=w146) -> (queue out=w168:refnum<queue>)  [unwired: 2 in, 2 out]
      n63 = Enqueue Element(queue=w161, element=w145) -> (queue out=w167:refnum<queue>)  [unwired: 2 in, 2 out]
      n64 = Enqueue Element(queue=w159, element=w144) -> (queue out=w164:refnum<queue>)  [unwired: 2 in, 2 out]
      n65 = Enqueue Element(queue=w158, element=w143) -> (queue out=w166:refnum<queue>)  [unwired: 2 in, 2 out]
      n66 = Enqueue Element(queue=w157, element=w142) -> (queue out=w165:refnum<queue>)  [unwired: 2 in, 2 out]
      n67 = Enqueue Element(queue=w156, element=w141) -> (queue out=w160:refnum<queue>)  [unwired: 2 in, 2 out]
      n68 = Index Array(array=w124) -> (element=w123:T14)  [unwired: 1 in]
      n69 = Unbundle By Name(w123) -> ("overflow"=→"overflow":i16)
      n70 = Get Queue Status(queue=w175) -> (queue out=w171:refnum<queue>, # elements in queue=→"queue depth" →"Queue depth":i32)  [unwired: 2 in, 6 out]
      n71 = Get Queue Status(queue=w174) -> (queue out=w170:refnum<queue>)  [unwired: 2 in, 7 out]
      n72 = Get Queue Status(queue=w169) -> (queue out=w155:refnum<queue>)  [unwired: 2 in, 7 out]
      n73 = Get Queue Status(queue=w168) -> (queue out=w154:refnum<queue>)  [unwired: 2 in, 7 out]
      n74 = Get Queue Status(queue=w167) -> (queue out=w153:refnum<queue>)  [unwired: 2 in, 7 out]
      n75 = Get Queue Status(queue=w164) -> (queue out=w152:refnum<queue>)  [unwired: 2 in, 7 out]
      n76 = Get Queue Status(queue=w166) -> (queue out=w151:refnum<queue>)  [unwired: 2 in, 7 out]
      n77 = Get Queue Status(queue=w165) -> (queue out=w150:refnum<queue>)  [unwired: 2 in, 7 out]
      n78 = Get Queue Status(queue=w160) -> (queue out=w149:refnum<queue>)  [unwired: 2 in, 7 out]
      n79 = Compound Arithmetic op=OR(w131, "stop", w198) -> (w199:bool)
      n80 = Compound Arithmetic op=OR(w199, "Apply Settings", w198) -> (w202:bool)
    }
    n81 = case shown="80000000" w93 {
      tunnel: [w212 u64 1 ("Down Sample Ratio")] -> w117
      tunnel: w94 -> [w212 _]
      frame Default {
      }
      frame -2147483648 {
        # "No DownSampling"
      }
    }
    n82 = Multiply(x=w117, y=w66) -> (x*y=→"DownSample Interval (sec)":dbl)
    n83 = call "PicoScope6000aStop.vi"("error in (no error)"=w90, "handle in"=w89) -> ("error out"=w91:errorcluster, "handle out"=w92:i16)  [unwired: 8 in]
    n84 = Unbundle By Name(w91) -> ("status"=w101:bool)
    n85 = Or(x=w100, y=w101) -> (x .or. y?=w99:bool)
  }
  n86 = call <vilib>:"Application Directory.vi"() -> ("Application Directory"=w27:path)
  n87 = Build Path(base path=w27, name or relative path="Data file") -> (appended path=w28:path)
  n88 = TDMS Open(6:FALSE ("disable buffering? (T)"), 7:enum16{"1.0", "2.0"}."1.0" ("file format version (2.0)"), 10:T8."create or replace" ("operation (0:open)"), 11:w28) -> (3:w33:refnum<k34>)  [unwired: 2 in, 1 out]
  n89 = Tick Count (ms)() -> (millisecond timer value=w35:u32)
  n90 = while {
    tunnel: w20 -> [w278]
    shift-right: [w270] -> _
    shift-left: w18 -> [w277]
    shift-right: [w272] -> _
    shift-left: w35 -> [w273]
    tunnel: w33 -> [w269]
    tunnel: [w268] -> w32
    shift-right: [w264] -> _
    shift-left: w18 -> [w266]
    shift-right: [w254] -> _
    shift-left: w18 -> [w255]
    shift-right: [w251] -> _
    shift-left: w18 -> [w252]
    shift-right: [w244] -> _
    shift-left: w18 -> [w249]
    shift-right: [w243] -> _
    shift-left: w18 -> [w248]
    shift-right: [w242] -> _
    shift-left: w18 -> [w247]
    shift-right: [w241] -> _
    shift-left: w18 -> [w246]
    shift-right: [w240] -> _
    shift-left: w18 -> [w245]
    tunnel: w16 -> [w225]
    tunnel: w15 -> [w224]
    tunnel: w14 -> [w223]
    tunnel: w13 -> [w222]
    tunnel: w12 -> [w221]
    tunnel: w11 -> [w220]
    tunnel: w10 -> [w219]
    tunnel: w9 -> [w218]
    stop <- w263 stop-if-true
    n91 = Dequeue Element(queue=w219) -> (element=w256:i16[], error out=w227:errorcluster)  [unwired: 2 in, 2 out]
    n92 = Dequeue Element(queue=w218) -> (element=w267:i16[], error out=w226:errorcluster)  [unwired: 2 in, 2 out]
    n93 = Dequeue Element(queue=w221) -> (element=w258:i16[], error out=w229:errorcluster)  [unwired: 2 in, 2 out]
    n94 = Dequeue Element(queue=w220) -> (element=w257:i16[], error out=w228:errorcluster)  [unwired: 2 in, 2 out]
    n95 = Dequeue Element(queue=w223) -> (element=w260:i16[], error out=w231:errorcluster)  [unwired: 2 in, 2 out]
    n96 = Dequeue Element(queue=w222) -> (element=w259:i16[], error out=w230:errorcluster)  [unwired: 2 in, 2 out]
    n97 = Dequeue Element(queue=w224) -> (element=w261:i16[], error out=w232:errorcluster)  [unwired: 2 in, 2 out]
    n98 = Tick Count (ms)() -> (millisecond timer value=w274:u32)
    n99 = Dequeue Element(queue=w225) -> (element=w262:i16[], error out=w233:errorcluster)  [unwired: 2 in, 2 out]
    n100 = Dequeue Element(queue=w278) -> (element=w279:i16[], error out=w234:errorcluster)  [unwired: 2 in, 2 out]
    n101 = Subtract(x=w274, y=w273) -> (x-y=w276:u32)
    n102 = case shown="No Error" w226 {
      tunnel: w266 -> [w310 w311]
      tunnel: [w309 w311] -> w265
      tunnel: w267 -> [w308 _]
      frame No Error {
        n103 = Build Array (concatenate)(w310, w308) -> (w309:i16[])
      }
      frame Error {
      }
    }
    n104 = case shown="No Error" w227 {
      tunnel: w245 -> [w282 w283]
      tunnel: [w281 w283] -> w235
      tunnel: w256 -> [w280 _]
      frame No Error {
        n105 = Build Array (concatenate)(w282, w280) -> (w281:i16[])
      }
      frame Error {
      }
    }
    n106 = case shown="No Error" w228 {
      tunnel: w246 -> [w286 w287]
      tunnel: [w285 w287] -> w236
      tunnel: w257 -> [w284 _]
      frame No Error {
        n107 = Build Array (concatenate)(w286, w284) -> (w285:i16[])
      }
      frame Error {
      }
    }
    n108 = Merge Errors(w234, w233, w232, w231, w230, w229, w228, w227, w226) -> (w217:errorcluster)
    n109 = case shown="No Error" w229 {
      tunnel: w247 -> [w290 w291]
      tunnel: [w289 w291] -> w237
      tunnel: w258 -> [w288 _]
      frame No Error {
        n110 = Build Array (concatenate)(w290, w288) -> (w289:i16[])
      }
      frame Error {
      }
    }
    n111 = case shown="No Error" w230 {
      tunnel: w248 -> [w294 w295]
      tunnel: [w293 w295] -> w238
      tunnel: w259 -> [w292 _]
      frame No Error {
        n112 = Build Array (concatenate)(w294, w292) -> (w293:i16[])
      }
      frame Error {
      }
    }
    n113 = case shown="No Error" w231 {
      tunnel: w249 -> [w298 w299]
      tunnel: [w297 w299] -> w239
      tunnel: w260 -> [w296 _]
      frame No Error {
        n114 = Build Array (concatenate)(w298, w296) -> (w297:i16[])
      }
      frame Error {
      }
    }
    n115 = case shown="No Error" w232 {
      tunnel: w252 -> [w302 w303]
      tunnel: [w301 w303] -> w250
      tunnel: w261 -> [w300 _]
      frame No Error {
        n116 = Build Array (concatenate)(w302, w300) -> (w301:i16[])
      }
      frame Error {
      }
    }
    n117 = case shown="No Error" w233 {
      tunnel: w255 -> [w306 w307]
      tunnel: [w305 w307] -> w253
      tunnel: w262 -> [w304 _]
      frame No Error {
        n118 = Build Array (concatenate)(w306, w304) -> (w305:i16[])
      }
      frame Error {
      }
    }
    n119 = case shown="No Error" w234 {
      tunnel: w277 -> [w385 w386]
      tunnel: [w384 w386] -> w271
      tunnel: w279 -> [w383 _]
      frame No Error {
        n120 = Build Array (concatenate)(w385, w383) -> (w384:i16[])
      }
      frame Error {
      }
    }
    n121 = Greater Or Equal?(x=w276, y=u32 1000) -> (x >= y?=w216:bool)
    n122 = Select(t=w274, s=w216, f=w273) -> (s? t:f=w272:u32)
    n123 = And(x=w216) -> (y=w214:errorcluster, x .and. y?=w215:bool)
    n124 = Unbundle By Name(w217, w214) -> ()
    n125 = case shown="True" w216 {
      tunnel: w271 -> [w322 w337]
      tunnel: [w322 w334] -> w270
      tunnel: w269 -> [w321 w325]
      tunnel: [w321 w324] -> w268
      tunnel: w265 -> [w320 w328]
      tunnel: [w320 w334] -> w264
      tunnel: [w319 w378] -> w263
      tunnel: w215 -> [w319 w378]
      tunnel: [w318 w334] -> w254
      tunnel: w253 -> [w318 w336]
      tunnel: [w317 w334] -> w251
      tunnel: w250 -> [w317 w335]
      tunnel: [w316 w334] -> w244
      tunnel: [w315 w334] -> w243
      tunnel: [w314 w334] -> w242
      tunnel: [w313 w334] -> w241
      tunnel: [w312 w334] -> w240
      tunnel: w239 -> [w316 w333]
      tunnel: w238 -> [w315 w332]
      tunnel: w237 -> [w314 w331]
      tunnel: w236 -> [w313 w330]
      tunnel: w235 -> [w312 w329]
      frame False {
      }
      frame True {
        w348 = u16 0 items=["unsigned binary", "offset binary", "2's complement"] ("data format (offset binary)")
        w334 = i16[] [] ("History Data")
        # "Once a second, save accumulated data to disk. Use LV TDMS file\nfor best performance; standard binary write also works."
        n126 = local read "Channels"() -> (w327:T1)
        n127 = local read "Max ADC value"() -> (w338:i16)
        n128 = Unbundle By Name(w327) -> ("Channel H Settings.Range"=w366:u32)
        n129 = Unbundle By Name(w327) -> ("Channel G Settings.Range"=w367:u32)
        n130 = Unbundle By Name(w327) -> ("Channel D Settings.Range"=w370:u32)
        n131 = Unbundle By Name(w327) -> ("Channel E Settings.Range"=w369:u32)
        n132 = Unbundle By Name(w327) -> ("Channel F Settings.Range"=w368:u32)
        n133 = Unbundle By Name(w327) -> ("Channel A Settings.Range"=w377:u32)
        n134 = Unbundle By Name(w327) -> ("Channel B Settings.Range"=w376:u32)
        n135 = Unbundle By Name(w327) -> ("Channel C Settings.Range"=w371:u32)
        n136 = call "PicoScopeAdcToVolts.vi"("Max_adc"=w338, "Range Index"=w366, "Data"=w329) -> ("Data"=w363:dbl[])
        n137 = call "PicoScopeAdcToVolts.vi"("Max_adc"=w338, "Range Index"=w377, "Data"=w337) -> ("Data"=w375:dbl[])
        n138 = call "PicoScopeAdcToVolts.vi"("Max_adc"=w338, "Range Index"=w367, "Data"=w330) -> ("Data"=w357:dbl[])
        n139 = call "PicoScopeAdcToVolts.vi"("Max_adc"=w338, "Range Index"=w369, "Data"=w332) -> ("Data"=w360:dbl[])
        n140 = call "PicoScopeAdcToVolts.vi"("Max_adc"=w338, "Range Index"=w368, "Data"=w331) -> ("Data"=w356:dbl[])
        n141 = call "PicoScopeAdcToVolts.vi"("Max_adc"=w338, "Range Index"=w370, "Data"=w333) -> ("Data"=w361:dbl[])
        n142 = call "PicoScopeAdcToVolts.vi"("Max_adc"=w338, "Range Index"=w376, "Data"=w336) -> ("Data"=w374:dbl[])
        n143 = call "PicoScopeAdcToVolts.vi"("Max_adc"=w338, "Range Index"=w371, "Data"=w335) -> ("Data"=w362:dbl[])
        n144 = local read "DownSample Interval (sec)"() -> (w339:dbl)
        n145 = Bundle(0, "DownSample Interval (sec)"=w339, "Data"=w375) -> (w373:T15)  [unwired: 1 in]
        n146 = Bundle(0, "DownSample Interval (sec)"=w339, "Data"=w374) -> (w372:T15)  [unwired: 1 in]
        n147 = Bundle(0, "DownSample Interval (sec)"=w339, "Data"=w362) -> (w355:T15)  [unwired: 1 in]
        n148 = Bundle(0, "DownSample Interval (sec)"=w339, "Data"=w360) -> (w353:T15)  [unwired: 1 in]
        n149 = Bundle(0, "DownSample Interval (sec)"=w339, "Data"=w356) -> (w352:T15)  [unwired: 1 in]
        n150 = Bundle(0, "DownSample Interval (sec)"=w339, "Data"=w357) -> (w351:T15)  [unwired: 1 in]
        n151 = Bundle(0, "DownSample Interval (sec)"=w339, "Data"=w361) -> (w354:T15)  [unwired: 1 in]
        n152 = Bundle(0, "DownSample Interval (sec)"=w339, "Data"=w363) -> (w350:T15)  [unwired: 1 in]
        n153 = call-poly <vilib>:"Analog to Digital.vi"("data format (offset binary)"=w348, "full-scale range (pk-pk)"=256.0, "resolution (16 bit)"=8, "analog waveform"=w328) -> ("digital waveform"=w344:digitalwaveform)  [unwired: 4 in, 3 out]
        n154 = Build Array(w373, w372, w355, w354, w353, w352, w351, w350) -> (w323:T16)
        "Analog Channels" <- w323
        n155 = Bundle By Name("t0"=timestamp(0 s since 1904-01-01), "dt"=w339, "Y"=w344) -> (→"Port 0":digitalwaveform)  [unwired: 1 in]
        n156 = case shown="True" "Write to TDMS file" {
          tunnel: w325 -> [w379 w382]
          tunnel: [w379 w381] -> w324
          tunnel: w323 -> [_ w380]
          frame False {
          }
          frame True {
            n157 = call "PicoWriteTDMS.vi"("Analog Channels"=w380, "Refnum in"=w382) -> ("Refnum out"=w381:refnum<k34>)  [unwired: 8 in, 1 out]
          }
        }
      }
    }
  }
  n158 = flat-sequence {
    tunnel: w25 -> [w390]
    tunnel: w1 -> [w389]
    tunnel: w24 -> [w388]
    tunnel: w23 -> [w387]
    tunnel: w22 -> [w400]
    tunnel: w21 -> [w399]
    tunnel: w8 -> [w398]
    tunnel: w7 -> [w397]
    tunnel: w6 -> [w396]
    tunnel: w5 -> [w395]
    tunnel: w4 -> [w394]
    tunnel: w3 -> [w393]
    tunnel: w2 -> [w392]
    frame #0 {
      n159 = call "PicoScope6000aClose.vi"("error in (no error)"=w388, "handle in"=w387) -> ("error out"=w391:errorcluster)  [unwired: 8 in, 1 out]
      n160 = call "PicoReleaseMultiBuffers.vi"("error in (no error)"=w391, "Enabled array"=w390, "Data Pointers"=w389) -> ()  [unwired: 7 in, 2 out]
    }
    frame #1 {
      n161 = Release Queue(queue=w400) -> ()  [unwired: 2 in, 3 out]
      n162 = Release Queue(queue=w399) -> ()  [unwired: 2 in, 3 out]
      n163 = Release Queue(queue=w398) -> ()  [unwired: 2 in, 3 out]
      n164 = Release Queue(queue=w397) -> ()  [unwired: 2 in, 3 out]
      n165 = Release Queue(queue=w396) -> ()  [unwired: 2 in, 3 out]
      n166 = Release Queue(queue=w395) -> ()  [unwired: 2 in, 3 out]
      n167 = Release Queue(queue=w394) -> ()  [unwired: 2 in, 3 out]
      n168 = Release Queue(queue=w393) -> ()  [unwired: 2 in, 3 out]
      n169 = Release Queue(queue=w392) -> ()  [unwired: 2 in, 3 out]
    }
  }
  n170 = TDMS Close(11:w32) -> ()  [unwired: 1 in, 2 out]
